vi "VIH HelpGen - Image - Find Ctrl Area in Conpane Picture.vi"(6 "Conpane Image Data":T2, 8 "error in":errorcluster, 9 "Top Left":cluster{"Row":i32, "Column":i32}, 10 "Ctrl Attributes":T3[](array[typedef]), 11 "Conpane Ctrl Refnums":refnum<vi>[](array[refnum])) -> (0 "error out":errorcluster, 1 "Terminals Info":T1(array[cluster]), 3 "dup Conpane Ctrl Refnums":refnum<vi>[](array[refnum]), 4 "ALL FOUND":bool, 5 "Not Found":cluster{"Ctrl ID":string, "Conpane Idx":i32}[](array[cluster]))   [LabVIEW 2014]
doc: "::: VI Helpeks :::\nCopyright (c) 2000-2026 Konstantin Shifershteyn. All rights reserved."
uses:
  VIH HelpGen Typedef - Control Terminal Attributes Cluster.ctl
  <vilib>/picture/picture.llb/imagedata.ctl
panel:
  # "VI Helpeks\nCopyright (c) 2012-2026 Konstantin Shifershteyn"
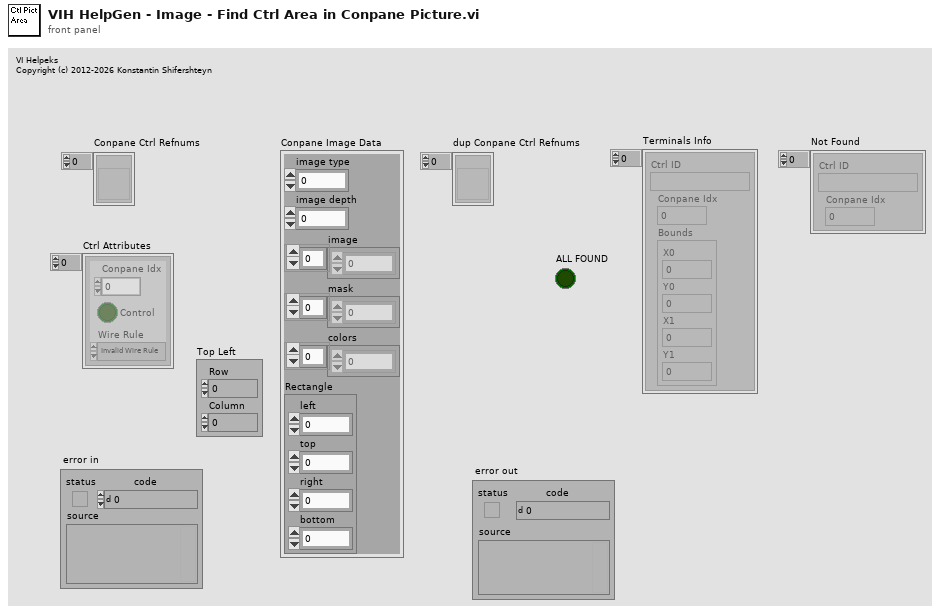
[diagram p1: front panel]
types:
  T1 = cluster{"Ctrl ID":string, "Conpane Idx":i32, "Bounds":cluster{"X0":i32, "Y0":i32, "X1":i32, "Y1":i32}}[]
  T2 = typedef "imagedata.ctl" = cluster{"image type":i32, "image depth":i32, "image":u8[], "mask":u8[], "colors":u32[], "Rectangle":cluster{"left":i16, "top":i16, "right":i16, "bottom":i16}}
  T3 = typedef "VIH HelpGen Typedef - Control Terminal Attributes Cluster.ctl" = cluster{"Conpane Idx":i32, "Control":bool, "Wire Rule":enum16{"Invalid Wire Rule", "Required", "Recommended", "Optional", "Dynamic Dispatch"}}
  T4 = cluster{"X0":i32, "Y0":i32, "X1":i32, "Y1":i32}[]
  T5 = cluster{"Ctrl Name":string, "Conpane Idx":i32, "Bounds":cluster{"X0":i32, "Y0":i32, "X1":i32, "Y1":i32}}[]
  T6 = cluster{"Conpane Idx":i32, "Control":bool, "Wire Rule":enum16{"Invalid Wire Rule", "Required", "Recommended", "Optional", "Dynamic Dispatch"}, "Conpane name":string, "Control ID":string, "Name image":u32[][]}[]
  T7 = cluster{"Control ID":string, "Conpane Idx":i32}[]
  T8 = cluster{"Control ID":string, "Conpane Idx":i32, "Bounds":cluster{"X0":i32, "Y0":i32, "X1":i32, "Y1":i32}}
  T9 = cluster{"Control ID":string, "Conpane Idx":i32, "Bounds":cluster{"X0":i32, "Y0":i32, "X1":i32, "Y1":i32}}[]
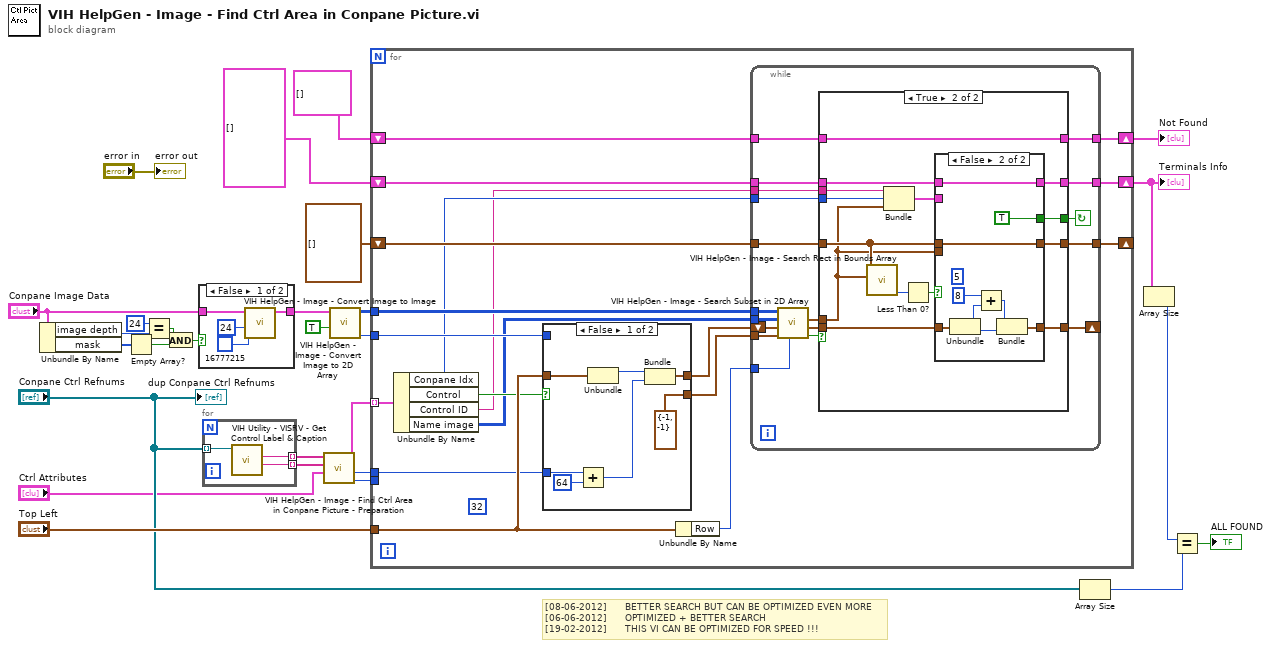
[diagram p0: block diagram]
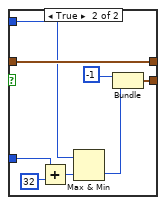
[diagram p3: hidden frame]
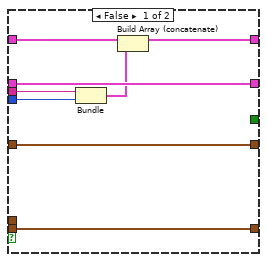
[diagram p4: hidden frame]
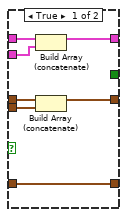
[diagram p5: hidden frame]
diagram:
  # "[08-06-2012]      BETTER SEARCH BUT CAN BE OPTIMIZED EVEN MORE\n[06-06-2012]      OPTIMIZED + BETTER SEARCH\n[19-02-2012]      THIS VI CAN BE OPTIMIZED FOR SPEED !!!"
  n1 = Unbundle By Name("Conpane Image Data") -> ("image depth"=w16:i32, "mask"=w14:u8[])
  n2 = Empty Array?(array=w14) -> (empty?=w13:bool)
  n3 = Equal?(x=24, y=w16) -> (x = y?=w12:bool)
  n4 = And(x=w12, y=w13) -> (x .and. y?=w11:bool)
  n5 = case shown="False" w11 {
    tunnel: "Conpane Image Data" -> [w32 w33]
    tunnel: [w31 w33] -> w18
    frame False {
      n6 = call "VIH HelpGen - Image - Convert Image to Image.vi"("BG Color (white)"=u32 16777215, "color depth (as source)"=24, "image data"=w32) -> ("image data out"=w31:T2)  [unwired: 8 in]
    }
    frame True {
    }
  }
  n7 = for {
    tunnel: "Conpane Ctrl Refnums" -> [w36] mode=indexing
    tunnel: [w35] -> w7 mode=indexing
    tunnel: [w34] -> w1 mode=indexing
    n8 = call "VIH Utility - VISRV - Get Control Label & Caption.vi"("Ctrl Refnum"=w36) -> ("Caption"=w34:string, "Label"=w35:string)  [unwired: 6 in, 3 out]
  }
  n9 = call "VIH HelpGen - Image - Find Ctrl Area in Conpane Picture - Preparation.vi"("Ctrl Attributes"="Ctrl Attributes", "Term Names"=w1, "Ctrl Labels"=w7) -> ("Max Column - Indicators"=w3:i32, "Max Column - Controls"=w4:i32, "Params"=w5:T6)  [unwired: 6 in]
  n10 = call "VIH HelpGen - Image - Convert Image to 2D Array.vi"("Black & White (F)"=TRUE, "Image Data"=w18) -> ("columns"=w9:i32, "Image 2D Array"=w28:u32[][])  [unwired: 7 in, 1 out]
  n11 = for {
    tunnel: w28 -> [w54]
    shift-right: [w52] -> w23
    shift-left: T5 [] -> [w53]
    shift-right: [w50] -> w24
    shift-left: cluster{"Ctrl Name":string, "Conpane Idx":i32}[] [] -> [w51]
    shift-right: [w48] -> _
    shift-left: T4 [] -> [w49]
    tunnel: "Top Left" -> [w46]
    tunnel: w9 -> [w43]
    tunnel: w5 -> [w42] mode=indexing
    tunnel: w4 -> [w37]
    tunnel: w3 -> [_]
    (unwired) 32 ("y")
    n12 = Unbundle By Name(w42) -> ("Conpane Idx"=w40:i32, "Control"=w41:bool, "Control ID"=w38:string, "Name image"=w39:u32[][])
    n13 = case shown="False" w41 {
      tunnel: w46 -> [w60 w69]
      tunnel: [w58 w69] -> w45
      tunnel: [cluster{i32, i32} {-1, -1} w67] -> w44
      tunnel: w43 -> [_ w64]
      tunnel: w37 -> [w57 w66]
      frame False {
        n14 = Add(x=w57, y=64) -> (x+y=w55:i32)
        n15 = Unbundle(w60) -> ("Row"=w59:i32)  [unwired: 1 out]
        n16 = Bundle("Row"=w59, w55) -> (w58:cluster{"Row":i32, i32})  [unwired: 1 in]
      }
      frame True {
        n17 = Add(x=w66, y=32) -> (x+y=w65:i32)
        n18 = Max & Min(x=w64, y=w65) -> (min(x,y)=w63:i32)  [unwired: 1 out]
        n19 = Bundle(-1, w63) -> (w67:cluster{i32, i32})  [unwired: 1 in]
      }
    }
    n20 = Unbundle By Name(w46) -> ("Row"=w47:i32)
    n21 = while {
      tunnel: w39 -> [w87]
      tunnel: w54 -> [w86]
      tunnel: w53 -> [w81]
      tunnel: [w80] -> w52
      tunnel: w40 -> [w79]
      tunnel: w38 -> [w78]
      shift-right: [w77] -> _
      shift-left: w45 -> [w76]
      tunnel: w51 -> [w75]
      tunnel: [w74] -> w50
      tunnel: w49 -> [w73]
      tunnel: [w72] -> w48
      tunnel: w47 -> [w71]
      tunnel: w44 -> [w70]
      stop <- w83 continue-if-true
      n22 = call "VIH HelpGen - Image - Search Subset in 2D Array.vi"("Min Row"=w71, "Finish Indices"=w70, "Start Indices"=w76, "2D subset"=w87, "Master 2D array"=w86) -> ("found"=w84:bool, "Found Indices"=w85:cluster{"Row":i32, "Column":i32}, "Bounds"=w82:cluster{"X0":i32, "Y0":i32, "X1":i32, "Y1":i32})  [unwired: 4 in]
      n23 = case shown="True" w84 {
        tunnel: w85 -> [w94 w103]
        tunnel: [_ w109] -> w83
        tunnel: w82 -> [_ w98]
        tunnel: w81 -> [w95 w108]
        tunnel: [w95 w107] -> w80
        tunnel: w79 -> [w92 w106]
        tunnel: w78 -> [w93 w104]
        tunnel: [w94 w102] -> w77
        tunnel: w75 -> [w90 w101]
        tunnel: [w89 w101] -> w74
        tunnel: w73 -> [w88 w99]
        tunnel: [w88 w100] -> w72
        frame False {
          n24 = Bundle("Control ID"=w93, "Conpane Idx"=w92) -> (w91:cluster{"Control ID":string, "Conpane Idx":i32})  [unwired: 1 in]
          n25 = Build Array (concatenate)(w90, w91) -> (w89:T7)
        }
        frame True {
          n26 = call "VIH HelpGen - Image - Search Rect in Bounds Array.vi"("Rect Bounds"=w98, "Rect array"=w99) -> ("Found Index"=w97:i32)  [unwired: 9 in]
          n27 = Bundle("Control ID"=w104, "Conpane Idx"=w106, "Bounds"=w98) -> (w105:T8)  [unwired: 1 in]
          n28 = Less Than 0?(x=w97) -> (x < 0?=w96:bool)
          n29 = case shown="False" w96 {
            tunnel: [_ TRUE] -> w109
            tunnel: w105 -> [w116 _]
            tunnel: w108 -> [w115 w124]
            tunnel: [w114 w124] -> w107
            tunnel: w103 -> [w113 w122]
            tunnel: [w113 w121] -> w102
            tunnel: w99 -> [w112 w123]
            tunnel: [w111 w123] -> w100
            tunnel: w98 -> [w110 _]
            frame True {
              n30 = Build Array (concatenate)(w115, w116) -> (w114:T9)
              n31 = Build Array (concatenate)(w112, w110) -> (w111:T4)
            }
            frame False {
              (unwired) 5 ("x")
              n32 = Unbundle(w122) -> ("Row"=w120:i32, "Column"=w118:i32)
              n33 = Add(x=8, y=w120) -> (x+y=w119:i32)
              n34 = Bundle(w119, "Column"=w118) -> (w121:cluster{i32, "Column":i32})  [unwired: 1 in]
            }
          }
        }
      }
    }
  }
  "Terminals Info" <- w23
  "Not Found" <- w24
  n35 = Array Size(array="Conpane Ctrl Refnums") -> (size(s)=w21:i32)
  n36 = Array Size(array=w23) -> (size(s)=w22:i32)
  n37 = Equal?(x=w22, y=w21) -> (x = y?=→"ALL FOUND":bool)
  "error out" <- "error in"
  "dup Conpane Ctrl Refnums" <- "Conpane Ctrl Refnums"
